vi "SV Sample.vi"(8 "error in (no error)":errorcluster) -> (0 "error out":errorcluster)   [LabVIEW 2025]
panel:
  out "timestamp":timestamp
  out "Value":dbl
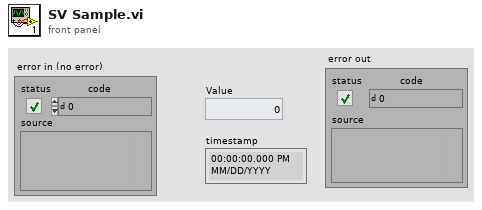
[diagram p1: front panel]
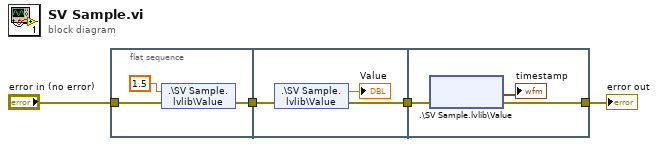
[diagram p0: block diagram]
diagram:
  n1 = flat-sequence {
    tunnel: "error in (no error)" -> [w6]
    tunnel: [w5] -> w1
    tunnel: [w8] -> w2
    tunnel: w1 -> [w9]
    tunnel: [w12] -> w3
    tunnel: w2 -> [w13]
    frame #0 {
      n2 = shared-variable ".\\SV Sample.lvlib\\Value"(1.5 ("Value"), error in=w6) -> (error out=w5:errorcluster)
    }
    frame #1 {
      n3 = shared-variable ".\\SV Sample.lvlib\\Value"(error in=w9) -> (→"Value":dbl, error out=w8:errorcluster)
    }
    frame #2 {
      n4 = shared-variable ".\\SV Sample.lvlib\\Value"(error in=w13) -> (error out=w12:errorcluster, →"timestamp":timestamp)  [unwired: 1 out]
    }
  }
  "error out" <- w3
